vi "Set Rig Config.vi"(8 "error in":errorcluster, 10 "Rig Config":T1, 11 "Rig in":refnum<class "Rig.lvclass">) -> (0 "error out":errorcluster, 3 "Rig out":refnum<class "Rig.lvclass">)   [LabVIEW 2026, in "Rig.lvclass"]
doc: "Stores the rig configuration (channels with unit and limits) in the rig object. Called by the executor before it launches the rig."
uses:
  Rig.lvclass
  Rig.lvclass/Rig.ctl
  Typedefs/Channel Definition.ctl
  Typedefs/Rig Config.ctl
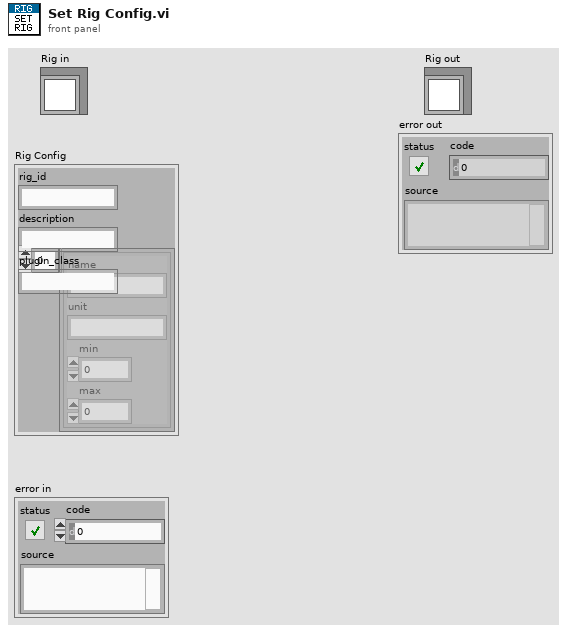
[diagram p1: front panel]
types:
  T1 = typedef "Rig Config.ctl" = cluster{"rig_id":string, "description":string, "plugin_class":string, "channels":T2[]}
  T2 = typedef "Channel Definition.ctl" = cluster{"name":string, "unit":string, "min":dbl, "max":dbl}
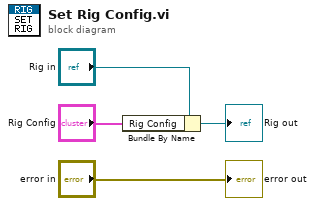
[diagram p0: block diagram]
diagram:
  n1 = Bundle By Name(cluster="Rig in", "Rig Config"="Rig Config") -> (→"Rig out":refnum<class "Rig.lvclass">)
  "error out" <- "error in"
